vi "Test Server Restart With Churning Client.vi"(8 "error in (no error)":errorcluster) -> (0 "error out":errorcluster)   [LabVIEW 2019, in "RemoteControl.ZMQ.Tests.lvclass"]
uses:
  RemoteControl.ZMQ.Tests.lvclass
  C:/Program Files/National Instruments/LabVIEW 2019/user.lib/LevyLab/RemoteControl/RemoteControl/RemoteControl.lvclass
  <userlib>/LevyLab/RemoteControl/RemoteControl/RemoteControl.lvclass/RemoteControl.ctl
  <vilib>/numeric/Random Number (Range) U64.vi
  422d38d7-e425-4e33-ac1b-a2d9845cf649.vi
  f0f0e852-f0d2-4d3c-8996-27ebcacf9f61.vi
  <vilib>/numeric/sub_Random U32.vi
  422d38d7-e425-4e33-ac1b-a2d9845cf649.vi/758215a8-1535-4d35-9ffd-7dac5027ed48.vi
  422d38d7-e425-4e33-ac1b-a2d9845cf649.vi/1f595430-411a-4d64-b909-f9957a72e8fe.vi
  f0f0e852-f0d2-4d3c-8996-27ebcacf9f61.vi/7c99dda3-071f-4f08-9a2c-ab661024165e.vi
  f0f0e852-f0d2-4d3c-8996-27ebcacf9f61.vi/57197ae9-7ae2-447f-86de-9249130d4f3d.vi
  <vilib>/Utility/Data Type/Get Type Information.vi
  <vilib>/JDP Science/JSONtext/JSON text to Variant.vi
  <vilib>/addons/_JKI Toolkits/Caraya/classes/Assert/Assert True.vi
  <vilib>/JDP Science/JSONtext/LVClass Serializer/JSONtext LVClass Serializer.lvclass
  <userlib>/LevyLab/RemoteControl/RemoteControl/RemoteControl.lvclass
  <vilib>/addons/_JKI Toolkits/Caraya/classes/Assert/Assert.lvclass
  <vilib>/addons/_JKI Toolkits/Caraya/classes/Test/Test.lvclass
panel:
  out "min time (ms)":u32
  out "max time (ms)":u32
  in  "stop 2":bool
  out "Equal?":bool[](array[boolean])
  out "Codes":i32[](array[numeric])
  in  "stop":bool
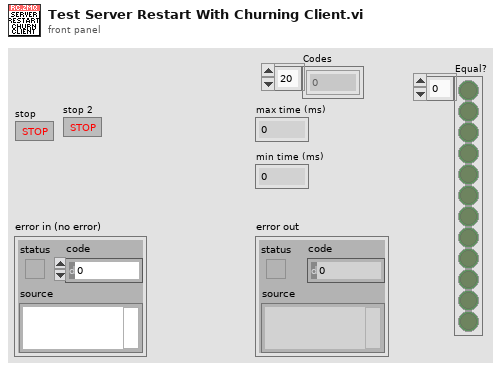
[diagram p1: front panel]
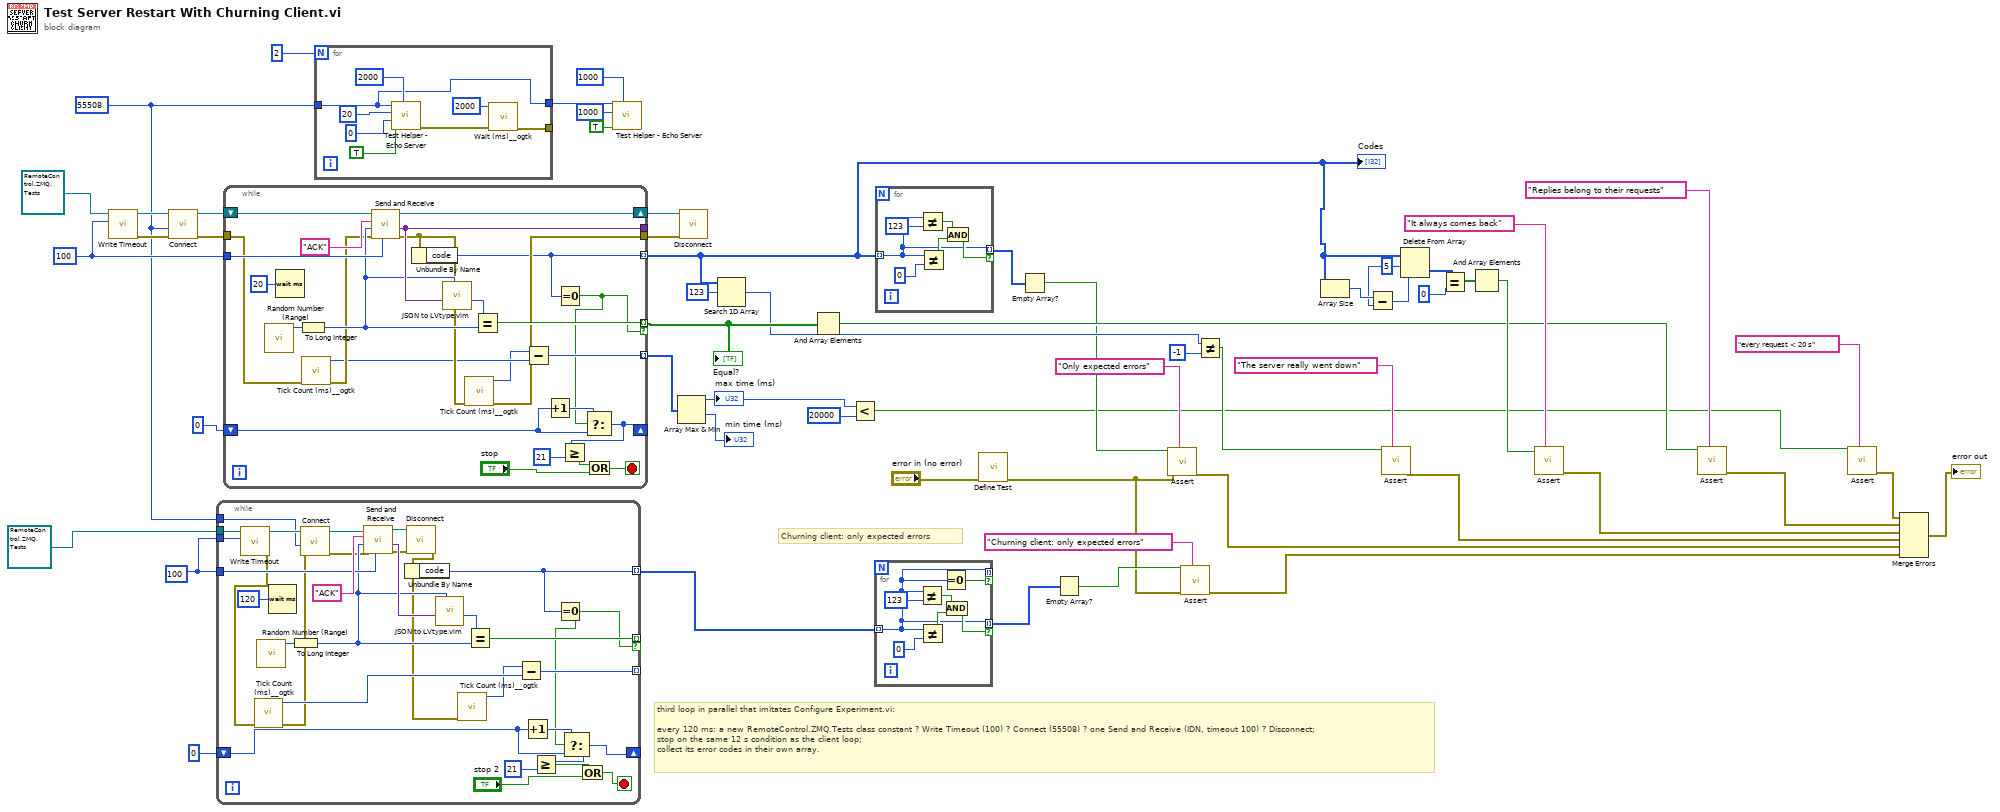
[diagram p0: block diagram]
diagram:
  w16 = 100 ("timeout in ms (100)")
  w30 = 5 ("length")
  w47 = 100 ("timeout in ms (100)")
  w9 = u16 55508 ("Port")
  # "Churning client: only expected errors"
  # "third loop in parallel that imitates Configure Experiment.vi:\n\nevery 120 ms: a new RemoteControl.ZMQ.Tests class constant ? Write Timeout (100) ? Connect (55508) ? one Send and Receive (IDN, timeout 100) ? Disconnect;\nstop on the same 12 s condition as the client loop;\ncollect its error codes in their own array."
  n1 = call <userlib>:"Write Timeout.vi"("timeout (ms) [500]"=w47, "RemoteControl in"=refnum<class "RemoteControl.ZMQ.Tests.lvclass"> refnum ("RemoteControl.ZMQ.Tests.lvclass")) -> ("error out"=w50:errorcluster, "RemoteControl out"=w49:refnum<class "RemoteControl.ZMQ.Tests.lvclass">)  [unwired: 8 in]
  n2 = call <userlib>:"Connect.vi"("error in (no error)"=w50, "Port"=w9, "RemoteControl in"=w49) -> ("error out"=w55:errorcluster, "RemoteControl out"=w57:refnum<class "RemoteControl.ZMQ.Tests.lvclass">)  [unwired: 7 in]
  n3 = while {
    tunnel: w16 -> [w86]
    tunnel: [w75] -> w15 mode=indexing
    tunnel: [w82] -> _ mode=indexing if=w62
    tunnel: [w79] -> _ mode=indexing
    tunnel: refnum<class "RemoteControl.ZMQ.Tests.lvclass"> refnum ("RemoteControl.ZMQ.Tests.lvclass") -> [w72]
    tunnel: w16 -> [w71]
    tunnel: w9 -> [w64]
    shift-right: [w58] -> _
    shift-left: 0 ("timeout in ms (100)") -> [w61]
    stop <- w76 stop-if-true
    n4 = call <userlib>:"Write Timeout.vi"("timeout (ms) [500]"=w71, "RemoteControl in"=w72) -> ("error out"=w70:errorcluster, "RemoteControl out"=w74:refnum<class "RemoteControl.ZMQ.Tests.lvclass">)  [unwired: 8 in]
    n5 = call <userlib>:"Tick Count (ms)__ogtk.vi"("error in (no error)"=w70) -> ("error out"=w69:errorcluster, "millisecond timer value"=w80:u32)  [unwired: 9 in]
    n6 = call-poly <vilib>:"Random Number (Range).vi"() -> ("number"=w88:u64)  [unwired: 11 in]
    n7 = Wait (ms)(milliseconds to wait=u32 120) -> ()  [unwired: 1 out]
    n8 = To Long Integer(number=w88) -> (32bit integer=w83:i32)
    n9 = call <userlib>:"Connect.vi"("error in (no error)"=w69, "Port"=w64, "RemoteControl in"=w74) -> ("error out"=w68:errorcluster, "RemoteControl out"=w73:refnum<class "RemoteControl.ZMQ.Tests.lvclass">)  [unwired: 7 in]
    n10 = call <userlib>:"Send and Receive.vi"("timeout (ms) [500]"=w86, "error in (no error)"=w68, "Data"=w83, "Command"="ACK", "RemoteControl in"=w73) -> ("error out"=w66:errorcluster, "Data out"=w85:variant, "RemoteControl out"=w67:refnum<class "RemoteControl.ZMQ.Tests.lvclass">)  [unwired: 3 in, 1 out]
    n11 = call <userlib>:"Disconnect.vi"("error in (no error)"=w66, "RemoteControl in"=w67) -> ("error out"=w65:errorcluster)  [unwired: 8 in, 1 out]
    n12 = Unbundle By Name(w65) -> ("code"=w75:i32)
    n13 = call "JSON to LVtype.vim"("type"=w83, "JSON Data in"=w85) -> ("Data out"=w84:i32)  [unwired: 8 in, 1 out]
    n14 = call <userlib>:"Tick Count (ms)__ogtk.vi"("error in (no error)"=w65) -> ("millisecond timer value"=w78:u32)  [unwired: 9 in, 1 out]
    n15 = Equal?(x=w84, y=w83) -> (x = y?=w82:bool)
    n16 = Subtract(x=w78, y=w80) -> (x-y=w79:u32)
    n17 = Increment(x=w61) -> (x+1=w63:i32)
    n18 = Equal To 0?(x=w75) -> (x = 0?=w62:bool)
    n19 = Select(t=w63, s=w62, f=w61) -> (s? t:f=w58:i32)
    n20 = Greater Or Equal?(x=w58, y=21) -> (x >= y?=w59:bool)
    n21 = Or(x=w59, y="stop 2") -> (x .or. y?=w76:bool)
  }
  n22 = while {
    tunnel: [w109] -> _
    tunnel: w47 -> [w110]
    shift-right: [w113] -> w56
    shift-left: w57 -> [w114]
    tunnel: w55 -> [w103]
    tunnel: [w101] -> w54
    tunnel: [w95] -> w28 mode=indexing
    tunnel: [w106] -> w40 mode=indexing if=w89
    tunnel: [w99] -> w8 mode=indexing
    shift-right: [w91] -> _
    shift-left: 0 ("timeout in ms (100)") -> [w94]
    stop <- w96 stop-if-true
    n23 = call-poly <vilib>:"Random Number (Range).vi"() -> ("number"=w112:u64)  [unwired: 11 in]
    n24 = Wait (ms)(milliseconds to wait=u32 20) -> ()  [unwired: 1 out]
    n25 = To Long Integer(number=w112) -> (32bit integer=w107:i32)
    n26 = call <userlib>:"Tick Count (ms)__ogtk.vi"("error in (no error)"=w103) -> ("error out"=w104:errorcluster, "millisecond timer value"=w100:u32)  [unwired: 9 in]
    n27 = call <userlib>:"Send and Receive.vi"("timeout (ms) [500]"=w110, "error in (no error)"=w104, "Data"=w107, "Command"="ACK", "RemoteControl in"=w114) -> ("error out"=w102:errorcluster, "Data out"=w109:variant, "RemoteControl out"=w113:refnum<class "RemoteControl.ZMQ.Tests.lvclass">)  [unwired: 3 in, 1 out]
    n28 = Unbundle By Name(w102) -> ("code"=w95:i32)
    n29 = call "JSON to LVtype.vim"("type"=w107, "JSON Data in"=w109) -> ("Data out"=w108:i32)  [unwired: 8 in, 1 out]
    n30 = call <userlib>:"Tick Count (ms)__ogtk.vi"("error in (no error)"=w102) -> ("error out"=w101:errorcluster, "millisecond timer value"=w98:u32)  [unwired: 9 in]
    n31 = Equal?(x=w108, y=w107) -> (x = y?=w106:bool)
    n32 = Subtract(x=w98, y=w100) -> (x-y=w99:u32)
    n33 = Increment(x=w94) -> (x+1=w93:i32)
    n34 = Equal To 0?(x=w95) -> (x = 0?=w89:bool)
    n35 = Select(t=w93, s=w89, f=w94) -> (s? t:f=w91:i32)
    n36 = Greater Or Equal?(x=w91, y=21) -> (x >= y?=w92:bool)
    n37 = Or(x=w92, y="stop") -> (x .or. y?=w96:bool)
  }
  "Codes" <- w28
  "Equal?" <- w40
  n38 = for {
    N: 2 -> [_]
    tunnel: w9 -> [w115]
    tunnel: [w117] -> _
    tunnel: [w115] -> w18
    n39 = call "Test Helper - Echo Server.vi"("idle timout"=u32 2000, "Answer?"=TRUE, "reply delay (ms)"=u32 0, "number of messages"=20, "port"=w115) -> ("error out"=w119:errorcluster)  [unwired: 5 in, 1 out]
    n40 = call <userlib>:"Wait (ms)__ogtk.vi"("error in (no error)"=w119, "milliseconds to wait"=u32 2000) -> ("error out"=w117:errorcluster)  [unwired: 8 in, 1 out]
  }
  n41 = call "Test Helper - Echo Server.vi"("idle timout"=u32 1000, "Answer?"=TRUE, "number of messages"=1000, "port"=w18) -> ()  [unwired: 6 in, 2 out]
  n42 = Array Max & Min(array=w8) -> (max value=w6:u32, min value=→"min time (ms)":u32)  [unwired: 2 out]
  "max time (ms)" <- w6
  n43 = call <userlib>:"Disconnect.vi"("error in (no error)"=w54, "RemoteControl in"=w56) -> ()  [unwired: 8 in, 2 out]
  n44 = Search 1D Array(1D array=w28, element=123) -> (index of element=w33:i32)  [unwired: 1 in]
  n45 = And Array Elements(Boolean array=w40) -> (logical AND=w39:bool)
  n46 = Less?(x=w6, y=u32 20000) -> (x < y?=w4:bool)
  n47 = for {
    tunnel: w15 -> [w124] mode=indexing
    tunnel: [w124] -> w13 mode=indexing if=w125
    tunnel: [w124] -> _ mode=indexing if=w123
    n48 = Not Equal?(x=w124, y=123) -> (x != y?=w127:bool)
    n49 = Not Equal?(x=w124, y=0) -> (x != y?=w126:bool)
    n50 = Equal To 0?(x=w124) -> (x = 0?=w123:bool)
    n51 = And(x=w127, y=w126) -> (x .and. y?=w125:bool)
  }
  n52 = for {
    tunnel: w28 -> [w130] mode=indexing
    tunnel: [w130] -> w35 mode=indexing if=w131
    n53 = Not Equal?(x=w130, y=123) -> (x != y?=w133:bool)
    n54 = Not Equal?(x=w130, y=0) -> (x != y?=w132:bool)
    n55 = And(x=w133, y=w132) -> (x .and. y?=w131:bool)
  }
  n56 = call <vilib>:"Define Test.vi"("error in (no error)"="error in (no error)") -> ("error out"=w11:errorcluster)  [unwired: 9 in, 1 out]
  n57 = Empty Array?(array=w35) -> (empty?=w32:bool)
  n58 = Empty Array?(array=w13) -> (empty?=w12:bool)
  n59 = call-poly <vilib>:"Assert.vi"("Label"="Only expected errors", "error in (no error)"=w11, "True?"=w32) -> ("error out"=w23:errorcluster)  [unwired: 7 in, 1 out]
  n60 = call-poly <vilib>:"Assert.vi"("Label"="Churning client: only expected errors", "error in (no error)"=w11, "True?"=w12) -> ("error out"=w10:errorcluster)  [unwired: 7 in, 1 out]
  n61 = Not Equal?(x=w33, y=-1) -> (x != y?=w36:bool)
  n62 = Array Size(array=w28) -> (size(s)=w31:i32)
  n63 = Subtract(x=w31, y=w30) -> (x-y=w29:i32)
  n64 = call-poly <vilib>:"Assert.vi"("Label"="The server really went down", "True?"=w36) -> ("error out"=w24:errorcluster)  [unwired: 8 in, 1 out]
  n65 = Delete From Array(array=w28, length=w30, index=w29) -> (deleted portion=w44:i32[])  [unwired: 1 out]
  n66 = Equal?(x=w44, y=0 ("length")) -> (x = y?=w42:bool[])
  n67 = And Array Elements(Boolean array=w42) -> (logical AND=w41:bool)
  n68 = call-poly <vilib>:"Assert.vi"("Label"="It always comes back", "True?"=w41) -> ("error out"=w25:errorcluster)  [unwired: 8 in, 1 out]
  n69 = call-poly <vilib>:"Assert.vi"("Label"="Replies belong to their requests", "True?"=w39) -> ("error out"=w26:errorcluster)  [unwired: 8 in, 1 out]
  n70 = call-poly <vilib>:"Assert.vi"("Label"="every request < 20 s", "True?"=w4) -> ("error out"=w27:errorcluster)  [unwired: 8 in, 1 out]
  n71 = Merge Errors(w27, w26, w25, w24, w23, w10) -> (→"error out":errorcluster)
